vi "Get Service Class Instances.vi"() -> (3 "service instances":refnum<class "ServiceBase.lvclass">[](array[class]))   [LabVIEW 2021, in "CanReaderCansub_server.lvlib"]
uses:
  CanReaderCansub_server.lvlib
  <vilib>/gRPC/LabVIEW gRPC Servicer/ServiceBase/ServiceBase.lvclass
  RPC Service/CanReaderCansub/CanReaderCansub.lvclass
  C:/Program Files/National Instruments/LabVIEW 2021/vi.lib/gRPC/LabVIEW gRPC Servicer/ServiceBase/ServiceBase.lvclass
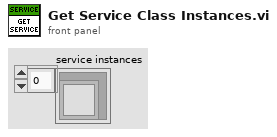
[diagram p1: front panel]
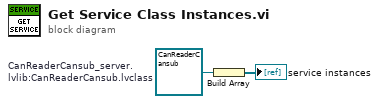
[diagram p0: block diagram]
diagram:
  w1 = refnum<class "CanReaderCansub.lvclass"> refnum  # CanReaderCansub_server.lvlib:CanReaderCansub.lvclass
  n1 = Build Array(w1) -> (→"service instances":refnum<class "CanReaderCansub.lvclass">[])
